vi "PicoScope5000aExampleRapidBlockBulkOverlapped.vi"() -> ()   [LabVIEW 2010]
uses:
  shared/PicoBuffers.ctl
  <vilib>/Waveform/DWDTOps.llb/DWDT Analog to Digital.vi
  PicoScope5000aLib/PicoScope5000aAnalogChannelSettings.ctl
  shared/Segment Range.ctl
  shared/Buffer and Transfer Settings.ctl
  shared/Acquisition Settings.ctl
  shared/nSegments.ctl
  PicoScope5000aLib/PicoScope5000aDigitalChannelSettings.ctl
panel:
  in  "roundFaster":bool=TRUE
  in  "timeIntervalRequested":dbl min=0.0 format="%#6_6p"
  in  "Write TDMS file":bool
  out "Total Requested Samples":u64
  out "overflow":i16[](array[numeric]) format="%06b"
  in  "Port 0 Settings":T1={"Enabled"=FALSE, "Logic Level"=9830} {"Logic Level" items=["1.5V TTL"=9830, "2.5V CMOS"=16383]}
  in  "Channel A Settings":T2={"Enabled"=TRUE, "Coupling"=1, "Range"=6, "Analogue Offset"=0.0, "Bandwidth Limit"=0} {"Bandwidth Limit" items=["Full", "20MHz"]; "Range" items=["10 mV", "20 mV", "50 mV", "100 mV", "200 mV", "500 mV", "1 V", "2 V", "5 V", "10 V", "20 V"]; "Coupling" items=["AC", "DC"]}
  in  "Trigger Settings":T3={"Trigger Enabled"=FALSE, "Trigger Source"=enum."Channel A", "Trigger Threshold (volts)"=0.0, "Trigger Direction"=2, "Trigger Delay (samples)"=0, "Auto Trigger Time (ms)"=1000} {"Trigger Direction" items=["Rising"=2, "Falling"=3]}
  out "USB 3.0 device on non-USB 3.0 Port":bool=TRUE
  out "USB Powered":bool=TRUE
  out "Device Info":T4={"Driver Version"="0", "USB Version"="0", "Hardware"="0", "Variant"="0", "Batch and Serial"="0", "Cal Date"="0", "Kernel Version"="0", "Digital HW Version"="0", "Analogue HW Version"="0", "MSO"=FALSE, "Number of channels"=0}
  out "Trigger Offsets":cluster{"Samples":u64, "Time (seconds)":sgl}[](array[cluster]) {"Time (seconds)" format="%#_5p"}
  in  "Stop Display":bool
  out "Capture Complete":bool
  in  "Run":bool
  in  "Display Buffer Index":i32
  in  "Segment Range":T5={"fromSegmentIndex"=0, "toSegmentIndex"=9} {"toSegmentIndex" format="%.4p"; "fromSegmentIndex" format="%.4p"}
  in  "nSegments":T6=10 format="%.4p"
  out "error out":errorcluster
  in  "Data file":path=path "PicoScope5000aExampleRapidBlock"
  in  "Buffer and Transfer Settings":T7={"startIndex"=0, "Samples"=1000000, "Down Sample Ratio"=1, "Down-Sample Mode"=0} {"Down-Sample Mode" items=["None"=0, "Aggregate"=1, "Decimate"=2, "Average"=4, "RAW none"=2147483648]; "Down Sample Ratio" step=1; "Samples" format="%_6p"}
  in  "Acquisition Settings":T8={"preTriggerSamples"=0, "postTriggerSamples"=1000000, "timebase"=0} {"postTriggerSamples" format="%_6p"; "preTriggerSamples" format="%_6p"}
  out "Properties Panel":T9 {"Max Total Capture Time Available (sec)" format="%.3p"; "Sample Frequency" format="%.6p"; "Sample Rate" format="%.3p"; "Max Samples Available" format="%_6p"; "Total Capture Time (sec)" format="%.3p"}
  out "Port 0":digitalwaveform(graph)={"t0"=timestamp(0 s since 1904-01-01), "dt"=8e-09, "Y"={"transitions"=[], "data"=[]}}
  in  "stop":bool
  out "Analog Channels":cluster{i32, sgl, "Data":dbl[]}[](graph)
  in  "Resolution":u32(ring) items=["8-bit"=0, "12-bit"=1, "14-bit"=2, "15-bit"=3, "16-bit"=4, "10-bit"=10]
  in  "Serial Number":string
  in  "Use Serial Number":bool
  in  "error in (no error)":errorcluster
  # "Number of\nSegments to Capture"
  # "Bit 0 = ChA"
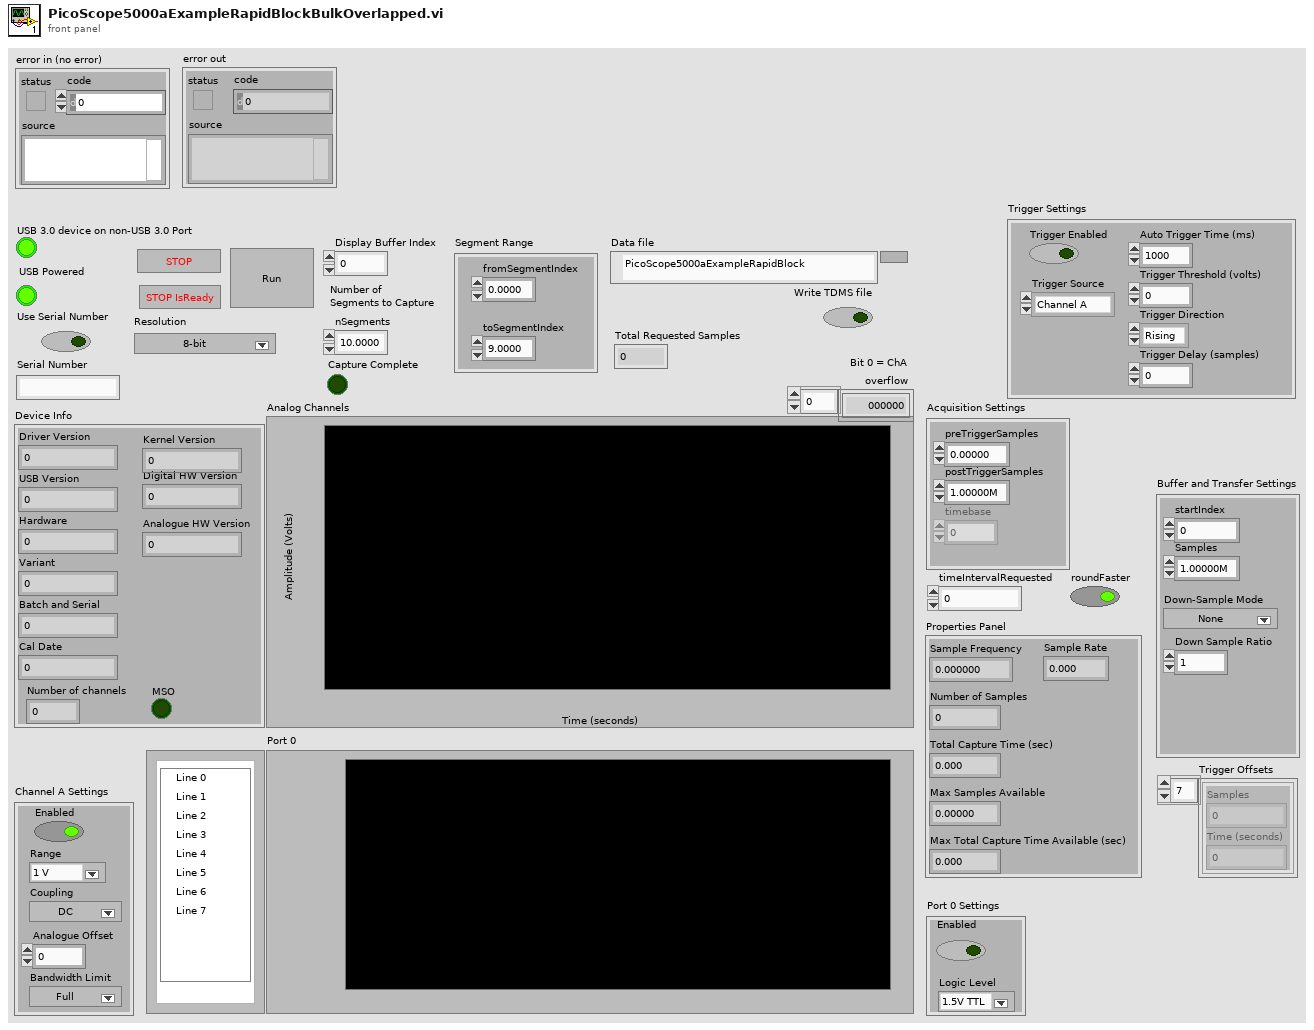
[diagram p1: front panel]
types:
  T1 = typedef "PicoScope5000aDigitalChannelSettings.ctl" = cluster{"Enabled":bool, "Logic Level":i16}
  T2 = typedef "PicoScope5000aAnalogChannelSettings.ctl" = cluster{"Enabled":bool, "Coupling":i16, "Range":u16, "Analogue Offset":sgl, "Bandwidth Limit":u32}
  T3 = cluster{"Trigger Enabled":bool, "Trigger Source":enum16{"Channel A", "Channel B", "Channel C", "Channel D", "Ext."}, "Trigger Threshold (volts)":dbl, "Trigger Direction":u16, "Trigger Delay (samples)":u32, "Auto Trigger Time (ms)":i16}
  T4 = cluster{"Driver Version":string, "USB Version":string, "Hardware":string, "Variant":string, "Batch and Serial":string, "Cal Date":string, "Kernel Version":string, "Digital HW Version":string, "Analogue HW Version":string, "MSO":bool, "Number of channels":i16}
  T5 = typedef "Segment Range.ctl" = cluster{"fromSegmentIndex":u64, "toSegmentIndex":u64}
  T6 = typedef "nSegments.ctl" = u64
  T7 = typedef "Buffer and Transfer Settings.ctl" = cluster{"startIndex":u64, "Samples":u64, "Down Sample Ratio":u64, "Down-Sample Mode":u32}
  T8 = typedef "Acquisition Settings.ctl" = cluster{"preTriggerSamples":u64, "postTriggerSamples":u64, "timebase":u32}
  T9 = cluster{"Sample Frequency":dbl, "Sample Rate":dbl, "Max Samples Available":u64, "Number of Samples":u64, "Total Capture Time (sec) ":dbl, "Max Total Capture Time Available (sec)":dbl}
  T10 = typedef "PicoBuffers.ctl" = cluster{"Max Buffer Pointers":u64[][][], "Min Buffer Pointers":u64[][][], "StreamingDataInfo":cluster{"Channel":u32, "Down-Sample Mode":u32, "PICO_DATA_TYPE":enum32{"PICO_INT8_T", "PICO_INT16_T", "PICO_INT32_T", "PICO_UINT32_T", "PICO_INT64_T", ""}, "Samples":i32, "bufferIndex":u64, "startIndex":i32, "overflow":i16}[][]}
  T11 = enum16{"open", "open or create", "create or replace", "create", "open (read-only)"}
  T12 = cluster{"Sample Frequency":sgl, "Sample Rate":sgl, "Max Samples Available":i32, "Number of Samples":u32, "Total Capture Time (sec) ":sgl, "Max Total Capture Time Available (sec)":sgl}
  T13 = cluster{"Channel A Buffer":i16[], "Channel B Buffer":i16[], "Channel C Buffer":i16[], "Channel D Buffer":i16[], "Channel E Buffer":i16[], "Channel F Buffer":i16[], "Channel G Buffer":i16[], "Channel H Buffer":i16[], "Port 0 Buffer":i16[], "Port 1 Buffer":i16[]}[]
  T14 = cluster{"Channel A Buffer":i16[], "Channel B Buffer":i16[], "Channel C Buffer":i16[], "Channel D Buffer":i16[], "Channel E Buffer":i16[], "Channel F Buffer":i16[], "Channel G Buffer":i16[], "Channel H Buffer":i16[], "Port 0 Buffer":i16[], "Port 1 Buffer":i16[]}
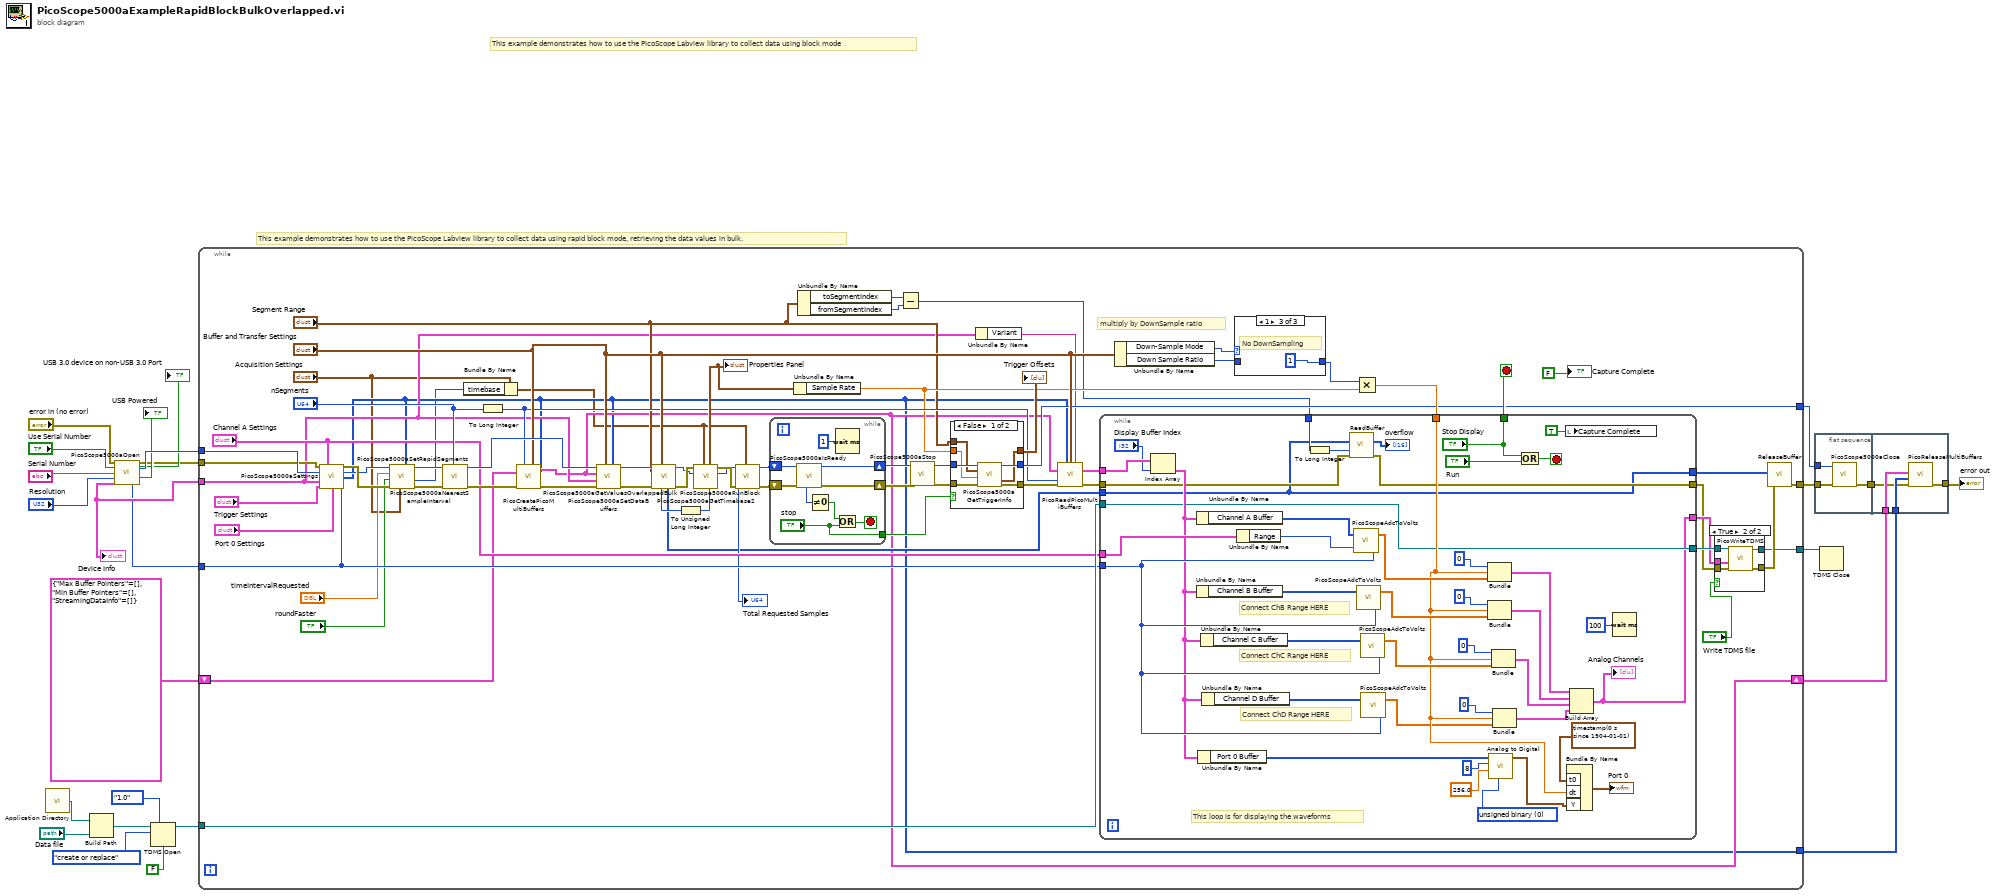
[diagram p0: block diagram]
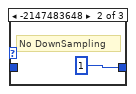
[diagram p5: hidden frame]
diagram:
  # "This example demonstrates how to use the PicoScope Labview library to collect data using rapid block mode, retrieving the data values in bulk."
  # "This example demonstrates how to use the PicoScope Labview library to collect data using block mode"
  n1 = call <vilib>:"Application Directory.vi"() -> ("Application Directory"=w19:path)
  n2 = Build Path(base path=w19, name or relative path="Data file") -> (appended path=w20:path)
  n3 = call "PicoScope5000aOpen.vi"("error in (no error)"="error in (no error)", "Serial Number"="Serial Number", "Use Serial Number"="Use Serial Number", "Resolution"="Resolution") -> ("USB 3.0 device on non-USB 3.0 Port"=→"USB 3.0 device on non-USB 3.0 Port":bool, "error out"=w8:errorcluster, "handle"=w25:i16, "USB Powered"=→"USB Powered":bool, "Device Info"=w12:T4, "Max ADC value"=w11:i16)  [unwired: 6 in]
  "Device Info" <- w12
  n4 = TDMS Open(6:FALSE ("disable buffering? (T)"), 7:enum16{"1.0", "2.0"}."1.0" ("file format version (2.0)"), 10:T11."create or replace" ("operation (0:open)"), 11:w20) -> (3:w17:refnum<k34>)  [unwired: 2 in, 1 out]
  n5 = while {
    tunnel: w25 -> [w64]
    tunnel: w11 -> [w58]
    tunnel: [w74] -> w6
    tunnel: [w31] -> w5
    tunnel: [w37] -> w18
    tunnel: w17 -> [w93]
    tunnel: w12 -> [w44]
    tunnel: w8 -> [w63]
    tunnel: [w51] -> w2
    shift-right: [w42] -> w4
    shift-left: T10 {"Max Buffer Pointers"=[], "Min Buffer Pointers"=[], "StreamingDataInfo"=[]} ("Data Pointers") -> [w43]
    stop <- w78 stop-if-true
    # "multiply by DownSample ratio"
    n6 = call "PicoScope5000aSettings.vi"("error in"=w63, "Channel A Settings"="Channel A Settings", "Port 0 Settings"="Port 0 Settings", "handle in"=w64, "Device Info"=w44, "Trigger Settings"="Trigger Settings", "Max ADC value"=w58) -> ("error out"=w35:errorcluster, "handle out"=w32:i16, "enabled array"=w31:i16[])  [unwired: 6 in]
    n7 = call "PicoScope5000aNearestSampleInterval.vi"("Enabled array"=w31, "Acquisition Settings"="Acquisition Settings", "error in (no error)"=w35, "roundFaster"="roundFaster", "timeIntervalRequested"="timeIntervalRequested", "handle in"=w32) -> ("error out"=w34:errorcluster, "timebase"=w27:u32, "handle out"=w33:i16)  [unwired: 2 in, 1 out]
    n8 = call "PicoScope5000aSetRapidSegments.vi"("nSegments"="nSegments", "error in (no error)"=w34, "handle in"=w33) -> ("error out"=w92:errorcluster, "handle out"=w91:i16)  [unwired: 6 in, 1 out]
    n9 = Bundle By Name(cluster="Acquisition Settings", "timebase"=w27) -> (w28:T8)
    n10 = To Long Integer(number="nSegments") -> (32bit integer=w60:i32)
    n11 = call "PicoCreatePicoMultiBuffers.vi"("Number of Buffers"=w60, "Buffer and Transfer Settings"="Buffer and Transfer Settings", "enabled array"=w31, "Data Pointers In"=w43, "error in (no error)"=w92) -> ("Data Pointers"=w42:T10, "error out"=w94:errorcluster)  [unwired: 9 in]
    n12 = call "PicoScope5000aSetDataBuffers.vi"("enabled array"=w31, "Buffer and Transfer Settings"="Buffer and Transfer Settings", "error in (no error)"=w94, "Device Info"=w44, "Data Pointers In"=w42, "handle in"=w91) -> ("error out"=w90:errorcluster, "handle out"=w89:i16)  [unwired: 4 in]
    n13 = call "PicoScope5000aGetValuesOverlappedBulk.vi"("Segment Range"="Segment Range", "Buffer and Transfer Settings"="Buffer and Transfer Settings", "error in (no error)"=w90, "handle in"=w89) -> ("error out"=w68:errorcluster, "handle out"=w67:i16, "Pointer to Overflow"=w50:u64[], "noOfSamples"=w53:u64)  [unwired: 4 in]
    n14 = To Unsigned Long Integer(number=w53) -> (unsigned 32bit integer=w52:u32)
    n15 = call "PicoScope5000aGetTimebase2.vi"("Number of Samples"=w52, "Acquisition Settings"=w28, "handle in"=w67, "error in (no error)"=w68) -> ("handle out"=w65:i16, "error out"=w66:errorcluster, "Properties Panel"=w84:T12)  [unwired: 5 in]
    "Properties Panel" <- w84
    n16 = call "PicoScope5000aRunBlock.vi"("Acquisition Settings"=w28, "error in (no error)"=w66, "handle in"=w65) -> ("error out"=w81:errorcluster, "handle out"=w80:i16, "Total Requested Samples"=→"Total Requested Samples":u64)  [unwired: 5 in, 1 out]
    n17 = while {
      shift-right: [w161] -> w72
      shift-left: w81 -> [w162]
      shift-right: [w160] -> w69
      shift-left: w80 -> [w159]
      tunnel: ["stop"] -> w57
      stop <- w155 stop-if-true
      n18 = call "PicoScope5000aIsReady.vi"("error in (no error)"=w162, "handle in"=w159) -> ("error out"=w161:errorcluster, "handle out"=w160:i16, "ready"=w157:i16)  [unwired: 7 in]
      n19 = Not Equal To 0?(x=w157) -> (x != 0?=w156:bool)
      n20 = Wait (ms)(milliseconds to wait=u32 1) -> ()  [unwired: 1 out]
      n21 = Or(x=w156, y="stop") -> (x .or. y?=w155:bool)
    }
    n22 = Unbundle By Name(w84) -> ("Sample Rate"=w56:sgl)
    n23 = Unbundle By Name("Segment Range") -> ("toSegmentIndex"=w48:u64, "fromSegmentIndex"=w47:u64)
    n24 = Subtract(x=w48, y=w47) -> (x-y=w45:u64)
    n25 = call "PicoScope5000aStop.vi"("error in (no error)"=w72, "handle in"=w69) -> ("error out"=w71:errorcluster, "handle out"=w70:i16)  [unwired: 8 in]
    n26 = case shown="False" w57 {
      tunnel: [w108 w109] -> w75
      tunnel: [w107 w110] -> w74
      tunnel: [w106 _] -> w73
      tunnel: w71 -> [w105 w109]
      tunnel: w70 -> [w104 w110]
      tunnel: "Segment Range" -> [w103 _]
      tunnel: w56 -> [w102 _]
      frame False {
        n27 = call "PicoScope5000aGetTriggerInfo.vi"("handle in"=w104, "Rapid Block Acquisition Settings"=w103, "Sample Rate"=w102, "error in"=w105) -> ("handle out"=w107:i16, "Trigger Offsets"=w106:cluster{u64, sgl}[], "error out"=w108:errorcluster)  [unwired: 8 in, 1 out]
      }
      frame True {
      }
    }
    "Trigger Offsets" <- w73
    n28 = Unbundle By Name(w44) -> ("Variant"=w55:string)
    n29 = call "PicoReadPicoMultiBuffers.vi"("enabled array"=w31, "Buffer and Transfer Settings"="Buffer and Transfer Settings", "Variant"=w55, "Data Pointers"=w42, "No of Buffers"=w60, "error in (no error)"=w75) -> ("MultiBuffers (Max or non-aggregated)"=w87:T13, "error out"=w79:errorcluster)  [unwired: 7 in, 1 out]
    n30 = Unbundle By Name("Buffer and Transfer Settings") -> ("Down-Sample Mode"=w85:u32, "Down Sample Ratio"=w86:u64)
    n31 = case shown="1" w85 {
      tunnel: [w163 u64 1 ("Down Sample Ratio") u64 1 ("Down Sample Ratio")] -> w82
      tunnel: w86 -> [w163 _ _]
      frame Default {
      }
      frame -2147483648 {
        # "No DownSampling"
      }
      frame 1 {
        # "No DownSampling"
      }
    }
    n32 = Multiply(x=w82, y=w56) -> (x*y=w83:sgl)
    n33 = while {
      tunnel: w58 -> [w127]
      tunnel: "Channel A Settings" -> [w153]
      tunnel: w87 -> [w126]
      tunnel: w83 -> [w128]
      tunnel: [w117] -> w39
      tunnel: w79 -> [w118]
      tunnel: ["Stop Display"] -> w78
      tunnel: w50 -> [w114]
      tunnel: [w114] -> w49
      tunnel: w45 -> [w115]
      tunnel: w93 -> [w112]
      tunnel: [w112] -> w41
      tunnel: [w111] -> w40
      stop <- w136 stop-if-true
      w145 = u16 0 items=["unsigned binary", "offset binary", "2's complement"] ("data format (offset binary)")
      # "This loop is for displaying the waveforms"
      # "Connect ChB Range HERE"
      # "Connect ChD Range HERE"
      # "Connect ChC Range HERE"
      n34 = Index Array(array=w126, index="Display Buffer Index") -> (element=w120:T14)
      n35 = Unbundle By Name(w120) -> ("Channel A Buffer"=w121:i16[])
      n36 = Unbundle By Name(w120) -> ("Channel B Buffer"=w150:i16[])
      n37 = Unbundle By Name(w120) -> ("Port 0 Buffer"=w143:i16[])
      n38 = Unbundle By Name(w120) -> ("Channel C Buffer"=w132:i16[])
      n39 = Unbundle By Name(w120) -> ("Channel D Buffer"=w124:i16[])
      n40 = Unbundle By Name(w153) -> ("Range"=w122:u16)
      n41 = To Long Integer(number=w115) -> (32bit integer=w119:i32)
      n42 = call "ReadBuffer.vi"("Pointer and BufferSize"=w114, "Buffer size"=w119, "error in (no error)"=w118) -> ("Output Array"=→"overflow":i16[], "error out"=w117:errorcluster)  [unwired: 11 in]
      n43 = call "PicoScopeAdcToVolts.vi"("Max_adc"=w127, "Range Index"=w122, "Data"=w121) -> ("Data"=w139:dbl[])
      n44 = call "PicoScopeAdcToVolts.vi"("Max_adc"=w127, "Data"=w150) -> ("Data"=w149:dbl[])  [unwired: 1 in]
      n45 = call "PicoScopeAdcToVolts.vi"("Max_adc"=w127, "Data"=w132) -> ("Data"=w131:dbl[])  [unwired: 1 in]
      n46 = call "PicoScopeAdcToVolts.vi"("Max_adc"=w127, "Data"=w124) -> ("Data"=w123:dbl[])  [unwired: 1 in]
      n47 = Bundle(0, w128, "Data"=w139) -> (w148:cluster{i32, sgl, "Data":dbl[]})  [unwired: 1 in]
      n48 = Bundle(0, w128, "Data"=w149) -> (w147:cluster{i32, sgl, "Data":dbl[]})  [unwired: 1 in]
      n49 = call-poly <vilib>:"Analog to Digital.vi"("data format (offset binary)"=w145, "full-scale range (pk-pk)"=256.0, "resolution (16 bit)"=8, "analog waveform"=w143) -> ("digital waveform"=w140:digitalwaveform)  [unwired: 4 in, 3 out]
      n50 = Bundle(0, w128, "Data"=w131) -> (w130:cluster{i32, sgl, "Data":dbl[]})  [unwired: 1 in]
      n51 = Bundle(0, w128, "Data"=w123) -> (w113:cluster{i32, sgl, "Data":dbl[]})  [unwired: 1 in]
      n52 = Or(x="Stop Display", y="Run") -> (x .or. y?=w136:bool)
      n53 = local write "Capture Complete"(TRUE ("Capture Complete")) -> ()
      n54 = Bundle By Name("t0"=timestamp(0 s since 1904-01-01), "dt"=w128, "Y"=w140) -> (→"Port 0":digitalwaveform)  [unwired: 1 in]
      n55 = Build Array(w148, w147, w130, w113) -> (w111:cluster{i32, sgl, "Data":dbl[]}[])
      "Analog Channels" <- w111
      n56 = Wait (ms)(milliseconds to wait=u32 100) -> ()  [unwired: 1 out]
    }
    n57 = case shown="True" "Write TDMS file" {
      tunnel: w41 -> [w95 w101]
      tunnel: w40 -> [_ w100]
      tunnel: w39 -> [w96 w99]
      tunnel: [w96 w98] -> w38
      tunnel: [w95 w97] -> w37
      frame False {
      }
      frame True {
        n58 = call "PicoWriteTDMS.vi"("error in (no error)"=w99, "Analog Channels"=w100, "Refnum in"=w101) -> ("error out"=w98:errorcluster, "Refnum out"=w97:refnum<k34>)  [unwired: 7 in]
      }
    }
    n59 = call "ReleaseBuffer.vi"("error in (no error)"=w38, "Pointer and BufferSize"=w49) -> ("error out"=w51:errorcluster)  [unwired: 9 in]
    "Capture Complete" <- FALSE ("Capture Complete")
  }
  n60 = flat-sequence {
    tunnel: w6 -> [w168]
    tunnel: w2 -> [w167]
    tunnel: [w166] -> w1
    tunnel: w5 -> [w172]
    tunnel: w4 -> [w171]
    tunnel: [w170] -> w3
    tunnel: w1 -> [w169]
    frame #0 {
      n61 = call "PicoScope5000aClose.vi"("error in (no error)"=w167, "handle in"=w168) -> ("error out"=w166:errorcluster)  [unwired: 8 in, 1 out]
    }
    frame #1 {
      n62 = call "PicoReleaseMultiBuffers.vi"("error in (no error)"=w169, "Enabled array"=w172, "Data Pointers"=w171) -> ("error out"=w170:errorcluster)  [unwired: 7 in, 1 out]
    }
  }
  n63 = TDMS Close(11:w18) -> ()  [unwired: 1 in, 2 out]
  "error out" <- w3
